vi "GenOneOf_Set_Accessor.vi"(7 "application reference":refnum<vi>, 8 "error in (no error)":errorcluster, 10 "message element metadata":T1, 11 "path":path) -> (0 "error out":errorcluster)   [LabVIEW 2019, in "gRPC Template Creation Utility.lvlib"]
uses:
  gRPC Template Creation Utility.lvlib
  TypeDefs/Message Element Metadata (Scripting).ctl
  TypeDefs/Message Element Type.ctl
  <vilib>/Utility/traverseref.llb/TRef TravTarget.ctl
  <vilib>/Utility/traverseref.llb/VI Scripting - Traverse.lvlib
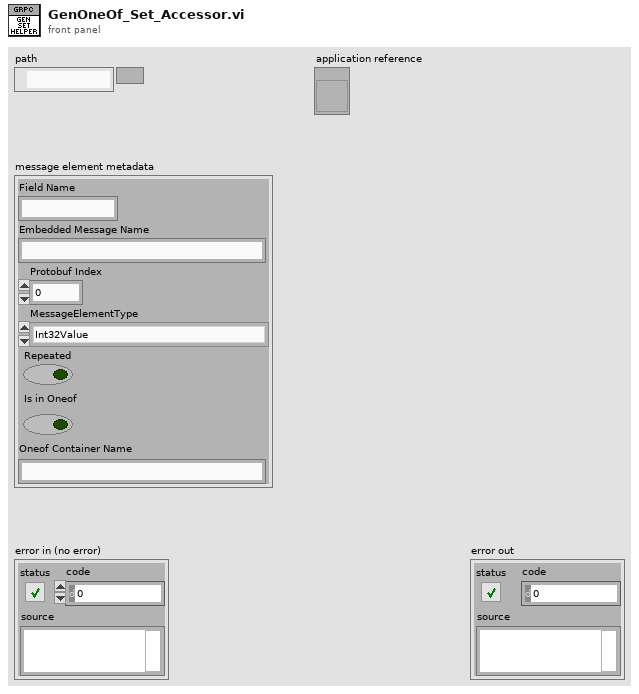
[diagram p1: front panel]
types:
  T1 = typedef "gRPC Template Creation Utility.lvlib/Message Element Metadata (Scripting).ctl" = cluster{"Field Name":string, "Embedded Message Name":string, "Protobuf Index":i32, "MessageElementType":T2, "Repeated":bool, "Is in Oneof":bool, "Oneof Container Name":string}
  T2 = typedef "gRPC Template Creation Utility.lvlib/Message Element Type.ctl" = enum32{"Int32Value", "FloatValue", "DoubleValue", "BoolValue", "StringValue", "MessageValue", "Int64Value", "UInt32Value", "UInt64Value", "EnumValue", "Bytes", "Fixed64", "Fixed32", "SFixed64", "SFixed32", "SInt64", "SInt32"}
  T3 = typedef "TRef TravTarget.ctl" = enum16{"FP", "BD", "Other"}
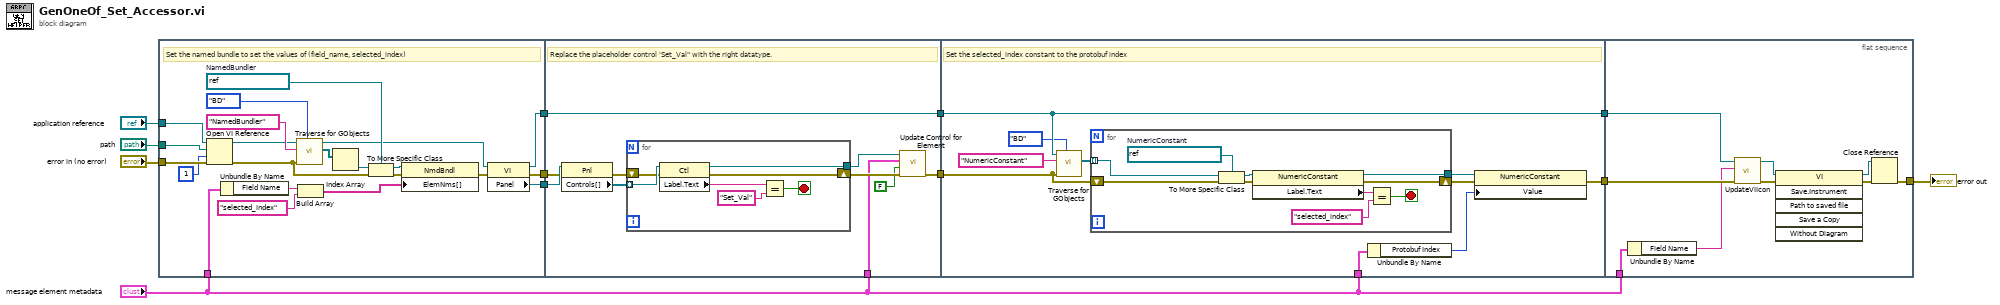
[diagram p0: block diagram]
diagram:
  n1 = flat-sequence {
    tunnel: "error in (no error)" -> [w34]
    tunnel: "path" -> [w27]
    tunnel: [w16] -> w12
    tunnel: [w23] -> w11
    tunnel: [w20] -> w10
    tunnel: "application reference" -> [w15]
    tunnel: "message element metadata" -> [w14]
    tunnel: w12 -> [w44]
    tunnel: w11 -> [w41]
    tunnel: w10 -> [w40]
    tunnel: [w44] -> w9
    tunnel: [w37] -> w8
    tunnel: "message element metadata" -> [w35]
    tunnel: w9 -> [w59]
    tunnel: w8 -> [w56]
    tunnel: [w59] -> w4
    tunnel: [w60] -> w3
    tunnel: "message element metadata" -> [w52]
    tunnel: [w78] -> w7
    tunnel: w4 -> [w74]
    tunnel: w3 -> [w77]
    tunnel: "message element metadata" -> [w73]
    frame #0 {
      w30 = refnum<vi> refnum  # NamedBundler
      # "Set the named bundle to set the values of (field_name, selected_index)"
      n2 = Open VI Reference(application reference (local)=w15, vi path=w27, options=1, error in (no error)=w34) -> (vi reference=w18:refnum<vi>, error out=w26:errorcluster)  [unwired: 2 in]
      n3 = Unbundle By Name(w14) -> ("Field Name"=w13:string)
      n4 = call <vilib>:"Traverse for GObjects.vi"("Traverse Target"=TRef_TravTarget."BD", "error in (no error)"=w26, "Class Name"="NamedBundler", "VI Refnum"=w18) -> ("References"=w31:refnum<vi>[], "dup VI Refnum"=w17:refnum<vi>)  [unwired: 4 in, 2 out]
      n5 = Build Array(w13, "selected_index" ("element")) -> (w28:string[])
      n6 = Index Array(array=w31) -> (element=w29:refnum<vi>)  [unwired: 1 in]
      n7 = To More Specific Class(target class=w30, reference=w29, error in=w26) -> (specific class reference=w24:refnum<vi>, error out=w22:errorcluster)
      n8 = property class="NmdBndl"(reference=w24, error in=w22, "ElemNms[]"=w28) -> (error out=w21:errorcluster)  [unwired: 1 out]
      n9 = property class="VI"(reference=w17, error in=w21) -> (reference out=w16:refnum<vi>, error out=w20:errorcluster, "Panel"=w23:refnum<vi>)
    }
    frame #1 {
      # "Replace the placeholder control 'Set_Val\" with the right datatype."
      n10 = property class="Pnl"(reference=w41, error in=w40) -> (error out=w43:errorcluster, "Controls[]"=w42:refnum<vi>[])  [unwired: 1 out]
      n11 = for {
        tunnel: w42 -> [w51] mode=indexing
        tunnel: [w47] -> w39
        shift-right: [w45] -> w38
        shift-left: w43 -> [w46]
        stop <- w48 stop-if-true
        n12 = property class="Ctl"(reference=w51, error in=w46) -> (reference out=w47:refnum<vi>, error out=w45:errorcluster, "Label.Text"=w50:string)
        n13 = Equal?(x=w50, y="Set_Val") -> (x = y?=w48:bool)
      }
      n14 = call "Update Control for Element.vi"("error in (no error)"=w38, "indicator"=FALSE, "message element metadata"=w35, "control to update"=w39) -> ("error out"=w37:errorcluster)  [unwired: 7 in]
    }
    frame #2 {
      # "Set the selected_index constant to the protobuf index"
      n15 = call <vilib>:"Traverse for GObjects.vi"("Traverse Target"=TRef_TravTarget."BD", "error in (no error)"=w56, "Class Name"="NumericConstant", "VI Refnum"=w59) -> ("References"=w55:refnum<vi>[])  [unwired: 4 in, 3 out]
      n16 = for {
        tunnel: w55 -> [w65] mode=indexing
        shift-right: [w67] -> w61
        shift-left: w56 -> [w66]
        tunnel: [w68] -> w54
        stop <- w69 stop-if-true
        w63 = refnum<vi> refnum  # NumericConstant
        n17 = To More Specific Class(target class=w63, reference=w65, error in=w66) -> (specific class reference=w64:refnum<vi>, error out=w62:errorcluster)
        n18 = property class="NumericConstant"(reference=w64, error in=w62) -> (reference out=w68:refnum<vi>, error out=w67:errorcluster, "Label.Text"=w71:string)
        n19 = Equal?(x=w71, y="selected_index") -> (x = y?=w69:bool)
      }
      n20 = Unbundle By Name(w52) -> ("Protobuf Index"=w53:i32)
      n21 = property class="NumericConstant"(reference=w54, error in=w61, "Value"=w53) -> (error out=w60:errorcluster)  [unwired: 1 out]
    }
    frame #3 {
      n22 = Unbundle By Name(w73) -> ("Field Name"=w72:string)
      n23 = call "UpdateVIIcon.vi"("error in (no error)"=w77, "Method Name"=w72, "VI in"=w74) -> ("error out"=w76:errorcluster, "VI out"=w75:refnum<vi>)  [unwired: 7 in]
      n24 = invoke class="VI" method="Save.Instrument"(reference=w75, error in=w76) -> (reference out=w79:refnum<vi>, error out=w80:errorcluster)  [unwired: 4 in, 4 out]
      n25 = Close Reference(reference=w79, error in (no error)=w80) -> (error out=w78:errorcluster)
    }
  }
  "error out" <- w7
